vi "refresh.vi"(8 "error in (no error)":errorcluster, 10 "Engine Configuration In":refnum<class "engine configuration.lvclass">, 11 "TDMS datalogger editor node In":refnum<class "TDMS datalogger editor node.lvclass">) -> (0 "error out":errorcluster, 2 "Engine Configuration Out":refnum<class "engine configuration.lvclass">, 3 "TDMS datalogger editor node Out":refnum<class "TDMS datalogger editor node.lvclass">)   [LabVIEW 2015, in "TDMS datalogger editor node.lvclass"]
uses:
  TDMS datalogger editor node.lvclass
  <vilib>/NI/Module Execution Interface/Engine Configuration/engine configuration.lvclass
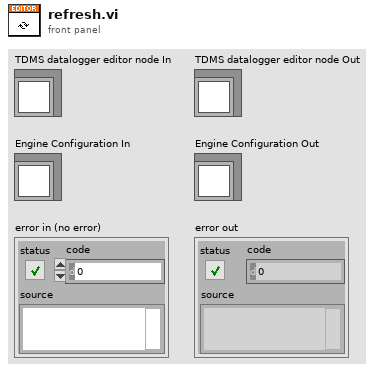
[diagram p1: front panel]
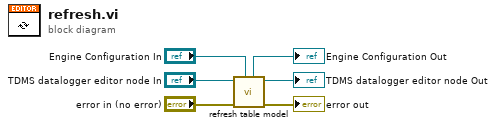
[diagram p0: block diagram]
diagram:
  n1 = call "refresh table model.vi"("engine configuration"="Engine Configuration In", "error in"="error in (no error)", "TDMS editor node"="TDMS datalogger editor node In") -> ("error out"=→"error out":errorcluster, "TDMS editor node out"=→"TDMS datalogger editor node Out":refnum<class "TDMS datalogger editor node.lvclass">, "engine configuration out"=→"Engine Configuration Out":refnum<class "engine configuration.lvclass">)  [unwired: 6 in]
